vi "Populate Single VI Help.vi"(6 "Show FP":bool, 7 "Force?(F)":bool, 8 "error in (no error)":errorcluster, 10 "VI Description":string, 11 "Path":path) -> (0 "error out":errorcluster)   [LabVIEW 2017, in "csmdoc.lvlib"]
uses:
  csmdoc.lvlib
  _Shared/CSM Shared.lvlib
  _tool/_file/csm-file-support.lvlib
  Communicable State Machine.lvlib
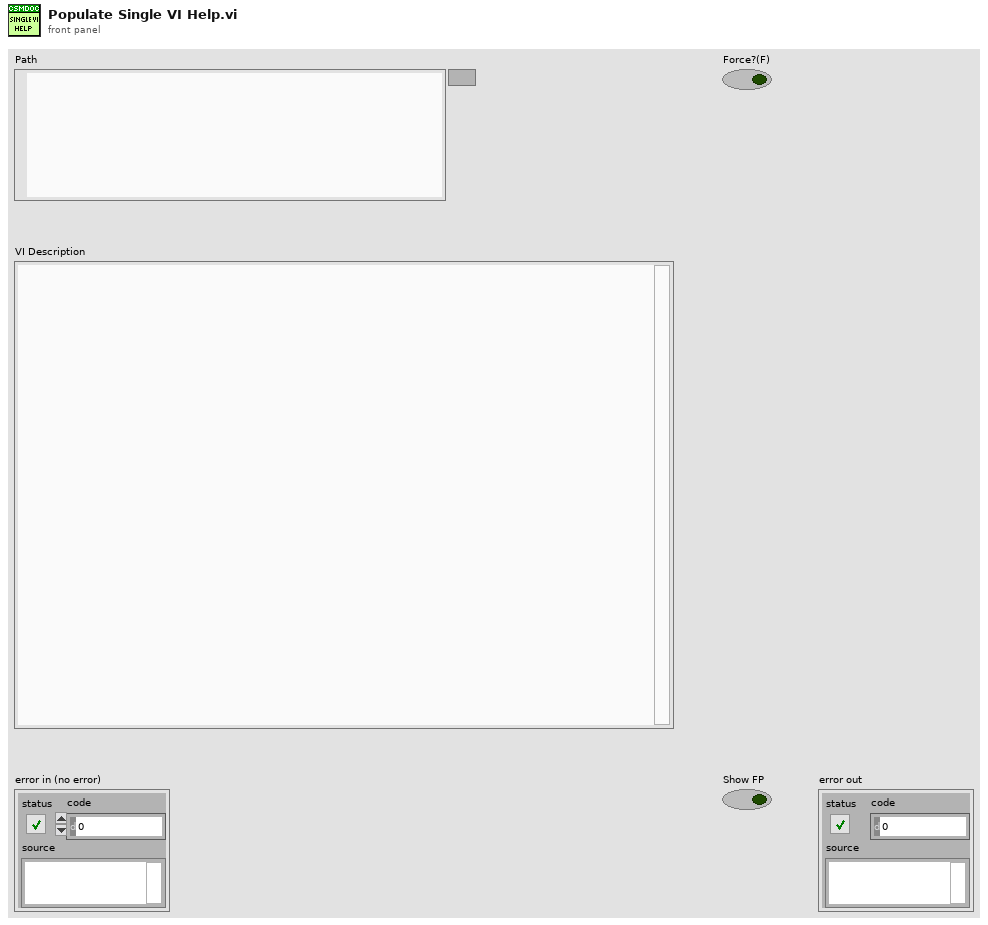
[diagram p1: front panel]
types:
  T1 = typedef "csmdoc.lvlib/DocElement.ctl" = cluster{"ID":string, "Content":string[], "SubIDs":string[], "Path":string[]}
  T2 = typedef "csmdoc.lvlib/DocNote.ctl" = cluster{"ID":string, "Content":string, "Type":string}
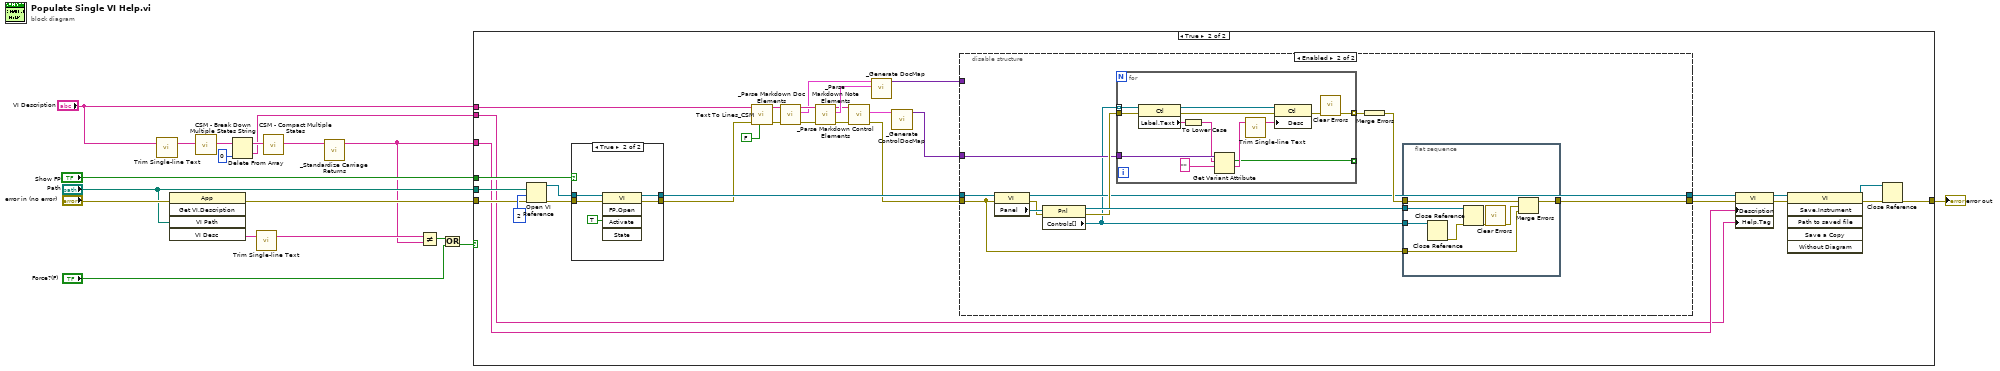
[diagram p0: block diagram]
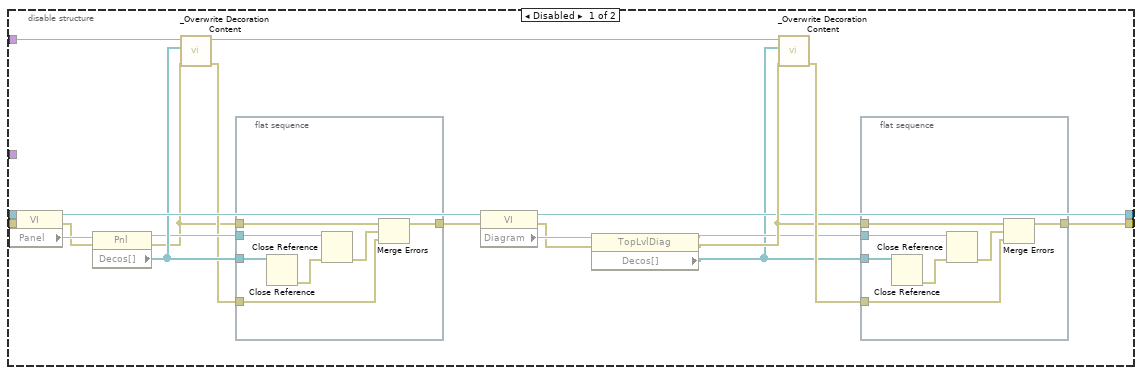
[diagram p3: hidden frame]
diagram:
  n1 = call "Trim Single-line Text.vi"("single-line text"="VI Description") -> ("trimed text"=w8:string)  [unwired: 2 in]
  n2 = invoke class="App" method="Get VI.Description"(error in="error in (no error)", "VI Path"="Path") -> (error out=w18:errorcluster, "VI Desc"=w13:string)  [unwired: 3 in, 3 out]
  n3 = call "CSM - Break Down Multiple States String.vi"("States"=w8) -> ("Multiple States"=w7:string[])  [unwired: 10 in]
  n4 = Delete From Array(array=w7, index=0) -> (deleted portion=w2:string, array with subset deleted=w5:string[])  [unwired: 1 in]
  n5 = call "Trim Single-line Text.vi"("single-line text"=w13) -> ("trimed text"=w17:string)  [unwired: 2 in]
  n6 = call "CSM - Compact Multiple States.vi"("Multiple States"=w5) -> ("States"=w3:string)  [unwired: 9 in]
  n7 = call "_Standardize Carriage Returns.vi"("States"=w3) -> ("trimed text"=w1:string)  [unwired: 10 in]
  n8 = Not Equal?(x=w17, y=w1) -> (x != y?=w10:bool)
  n9 = Or(x=w10, y="Force?(F)") -> (x .or. y?=w11:bool)
  n10 = case shown="True" w11 {
    tunnel: w18 -> [w19 w46]
    tunnel: "VI Description" -> [_ w31]
    tunnel: [w19 w43] -> w15
    tunnel: "Show FP" -> [_ w50]
    tunnel: "Path" -> [_ w42]
    tunnel: w1 -> [_ w21]
    tunnel: w2 -> [_ w20]
    frame False {
    }
    frame True {
      n11 = Open VI Reference(vi path=w42, options=2, error in (no error)=w46) -> (vi reference=w47:refnum<vi>, error out=w48:errorcluster)  [unwired: 3 in]
      n12 = case shown="True" w50 {
        tunnel: w48 -> [w118 w123]
        tunnel: w47 -> [w119 w122]
        tunnel: [w118 w121] -> w32
        tunnel: [w119 w120] -> w33
        frame False {
        }
        frame True {
          n13 = invoke class="VI" method="FP.Open"(reference=w122, error in=w123, "Activate"=TRUE ("Activate?")) -> (reference out=w120:refnum<vi>, error out=w121:errorcluster)  [unwired: 2 in, 3 out]
        }
      }
      n14 = call "Text To Lines_CSM.vi"("Remove Empty Lines? (T)"=FALSE ("Remove Empty Lines?(T)"), "error in (no error)"=w32, "String"=w31) -> ("error out"=w39:errorcluster, "Lines"=w40:string[])  [unwired: 7 in]
      n15 = call "_Parse Markdown Doc Elements.vi"("Error in"=w39, "Lines"=w40) -> ("Error out"=w37:errorcluster, "Array"=w36:T1[], "Lines (dup)"=w38:string[])  [unwired: 7 in]
      n16 = call "_Parse Markdown Note Elements.vi"("Error in"=w37, "Lines"=w38) -> ("Error out"=w25:errorcluster, "Array"=w35:T2[], "Lines (dup)"=w26:string[])  [unwired: 7 in]
      n17 = call "_Parse Markdown Control Elements.vi"("Error in"=w25, "Lines"=w26) -> ("Error out"=w24:errorcluster, "Array"=w23:T2[])  [unwired: 7 in, 1 out]
      n18 = call "_Generate DocMap.vi"("Array 2"=w35, "Array"=w36) -> ("Variant"=w34:variant)  [unwired: 9 in]
      n19 = call "_Generate ControlDocMap.vi"("Array"=w23) -> ("Variant"=w22:variant)  [unwired: 10 in]
      n20 = disable-structure shown="Enabled" {
        disable-tunnel: w24 -> [w68 w86]
        disable-tunnel: w34 -> [w63 _]
        disable-tunnel: w33 -> [w62 w95]
        disable-tunnel: [w53 w89] -> w30
        disable-tunnel: [w52 w90] -> w29
        disable-tunnel: w22 -> [_ w88]
        frame Disabled {
          n21 = property class="VI"(reference=w62, error in=w68) -> (reference out=w69:refnum<vi>, error out=w64:errorcluster, "Panel"=w70:refnum<vi>)
          n22 = property class="Pnl"(reference=w70, error in=w64) -> (reference out=w66:refnum<vi>, error out=w60:errorcluster, "Decos[]"=w67:refnum<vi>[])
          n23 = call "_Overwrite Decoration Content.vi"("error in (no error)"=w60, "Decos[]"=w67, "Variant in"=w63) -> ("error out"=w61:errorcluster, "Variant out"=w54:variant)  [unwired: 7 in]
          n24 = flat-sequence {
            tunnel: w67 -> [w84]
            tunnel: w66 -> [w83]
            tunnel: [w81] -> w65
            tunnel: w60 -> [w79]
            tunnel: w61 -> [w78]
            frame #0 {
              n25 = Close Reference(reference=w84) -> (error out=w82:errorcluster)  [unwired: 1 in]
              n26 = Close Reference(reference=w83, error in (no error)=w82) -> (error out=w80:errorcluster)
              n27 = Merge Errors(w79, w80, w78) -> (w81:errorcluster)
            }
          }
          n28 = property class="VI"(reference=w69, error in=w65) -> (reference out=w53:refnum<vi>, error out=w58:errorcluster, "Diagram"=w59:refnum<vi>)
          n29 = property class="TopLvlDiag"(reference=w59, error in=w58) -> (reference out=w55:refnum<vi>, error out=w56:errorcluster, "Decos[]"=w51:refnum<vi>[])
          n30 = call "_Overwrite Decoration Content.vi"("error in (no error)"=w56, "Decos[]"=w51, "Variant in"=w54) -> ("error out"=w57:errorcluster)  [unwired: 7 in, 1 out]
          n31 = flat-sequence {
            tunnel: w51 -> [w77]
            tunnel: w55 -> [w76]
            tunnel: [w74] -> w52
            tunnel: w56 -> [w72]
            tunnel: w57 -> [w71]
            frame #0 {
              n32 = Close Reference(reference=w77) -> (error out=w75:errorcluster)  [unwired: 1 in]
              n33 = Close Reference(reference=w76, error in (no error)=w75) -> (error out=w73:errorcluster)
              n34 = Merge Errors(w72, w73, w71) -> (w74:errorcluster)
            }
          }
        }
        frame Enabled {
          n35 = property class="VI"(reference=w95, error in=w86) -> (reference out=w89:refnum<vi>, error out=w85:errorcluster, "Panel"=w96:refnum<vi>)
          n36 = property class="Pnl"(reference=w96, error in=w85) -> (reference out=w94:refnum<vi>, error out=w91:errorcluster, "Controls[]"=w87:refnum<vi>[])
          n37 = for {
            tunnel: w87 -> [w117] mode=indexing
            tunnel: w91 -> [w116]
            tunnel: [w105] -> w93 mode=indexing
            tunnel: [w109] -> _ mode=indexing
            tunnel: w88 -> [w107]
            n38 = property class="Ctl"(reference=w117, error in=w116) -> (reference out=w115:refnum<vi>, error out=w114:errorcluster, "Label.Text"=w112:string)
            n39 = To Lower Case(string=w112) -> (all lower case string=w106:string)
            n40 = Get Variant Attribute(Variant=w107, name=w106, default value (empty Variant)="" ("regular expression")) -> (found=w109:bool, value=w110:string)  [unwired: 1 in, 2 out]
            n41 = call "Trim Single-line Text.vi"("single-line text"=w110) -> ("trimed text"=w108:string)  [unwired: 2 in]
            n42 = property class="Ctl"(reference=w115, error in=w114, "Desc"=w108) -> (error out=w113:errorcluster)  [unwired: 1 out]
            n43 = call <vilib>:"Clear Errors.vi"("error in (no error)"=w113) -> ("error out"=w105:errorcluster)  [unwired: 5 in, 1 out]
          }
          n44 = Merge Errors(w93) -> (w92:errorcluster)
          n45 = flat-sequence {
            tunnel: w87 -> [w104]
            tunnel: w94 -> [w103]
            tunnel: [w101] -> w90
            tunnel: w92 -> [w99]
            tunnel: w86 -> [w98]
            frame #0 {
              n46 = Close Reference(reference=w104) -> (error out=w102:errorcluster)  [unwired: 1 in]
              n47 = Close Reference(reference=w103, error in (no error)=w102) -> (error out=w100:errorcluster)
              n48 = call <vilib>:"Clear Errors.vi"("error in (no error)"=w100) -> ("error out"=w97:errorcluster)  [unwired: 5 in, 1 out]
              n49 = Merge Errors(w99, w97, w98) -> (w101:errorcluster)
            }
          }
        }
      }
      n50 = property class="VI"(reference=w30, error in=w29, "Description"=w21, "Help.Tag"=w20) -> (reference out=w27:refnum<vi>, error out=w28:errorcluster)
      n51 = invoke class="VI" method="Save.Instrument"(reference=w27, error in=w28) -> (reference out=w44:refnum<vi>, error out=w45:errorcluster)  [unwired: 4 in, 4 out]
      n52 = Close Reference(reference=w44, error in (no error)=w45) -> (error out=w43:errorcluster)
    }
  }
  "error out" <- w15
